vi "[ce] CalcExpress - Not a CE InstanceRef.vi"(0 "CE InstanceRef":T1) -> (1 "dynamically opened":bool, 2 "not a CE Instance":bool)   [LabVIEW 2021]
doc: "This VI validates a reference to a CalcExpress instance context. Refer to the VI help for more details.\n\n<B>not a CE Instance</B> indicator contains TRUE if <B>CE InstanceRef</B> is not a valid CalcExpress instance context reference.\n\n<B>dynamically opened</B> indicator contains TRUE if <B>CE InstanceRef</B> is valid and refers to a dynamically created CalcExpress instance context.\n\nFor more information, see help for this VI.\n\n::: CalcExpress Toolkit :::\nCopyright (c) 2000-2026 Konstantin Shifershteyn. All rights reserved."
uses:
  cetypes.llb/CalcExpress Instance RefNum.ctl
  cersrc/celveng32.dll
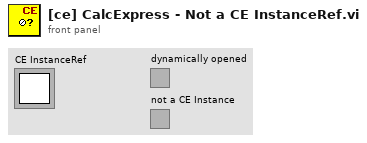
[diagram p1: front panel]
types:
  T1 = typedef "CalcExpress Instance RefNum.ctl" = refnum<k1>
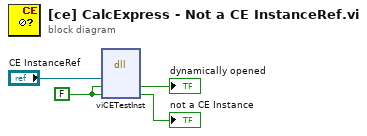
[diagram p0: block diagram]
diagram:
  w3 = FALSE ("not a CE Instance")
  n1 = dll-call lib="C:/LV Projects/CalcExpress 40 LV2021/vi.lib/addons/CalcExpress/cersrc/celveng*.dll" fn="viCETestInst"("iRef"="CE InstanceRef", "fDyn"=w3, "erf"=w3) -> ("fDyn"=→"dynamically opened":bool, "erf"=→"not a CE Instance":bool)  [unwired: 5 in, 2 out]
